vi "Create.vi"(9 "Control Values":cluster{"Name":string, "Control Data":variant}[](array[cluster]), 10 "VI Name":string) -> (3 "Parametric VI Call Out":refnum<class "Parametric VI Call.lvclass">)   [LabVIEW 2020, in "Parametric VI Call.lvclass"]
uses:
  Parametric VI Call.lvclass
  Parametric VI Call.lvclass/Parametric VI Call.ctl
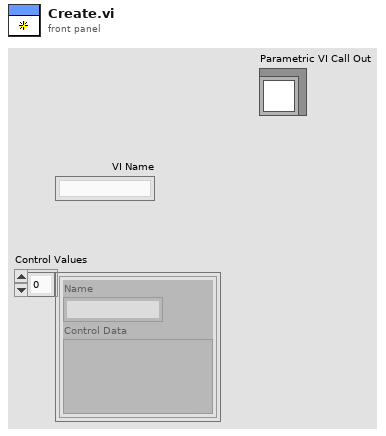
[diagram p1: front panel]
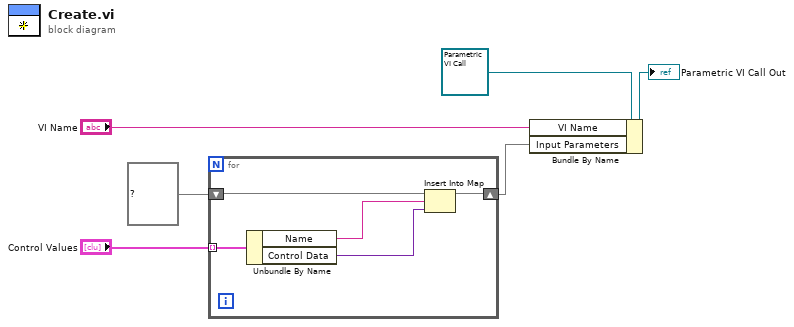
[diagram p0: block diagram]
diagram:
  n1 = for {
    shift-right: [w10] -> w1
    shift-left: map{string, variant} {} ("map") -> [w11]
    tunnel: "Control Values" -> [w9] mode=indexing
    n2 = Unbundle By Name(w9) -> ("Name"=w8:string, "Control Data"=w7:variant)
    n3 = Insert Into Map(map in=w11, key=w8, value=w7) -> (map out=w10:map{string, variant})  [unwired: 2 out]
  }
  n4 = Bundle By Name(cluster=refnum<class "Parametric VI Call.lvclass"> refnum ("Parametric VI Call"), "VI Name"="VI Name", "Input Parameters"=w1) -> (→"Parametric VI Call Out":refnum<class "Parametric VI Call.lvclass">)
